vi "Disconnect.vi"(8 "error in (no error)":errorcluster, 10 "Disconnection list in":string, 11 "Consumer in":refnum<class "Consumer.lvclass">) -> (0 "error out":errorcluster, 3 "Consumer out":refnum<class "Consumer.lvclass">)   [LabVIEW 2020, in "%DEVICE% Messaging.lvlib" / "Consumer.lvclass"]
uses:
  Consumer.lvclass
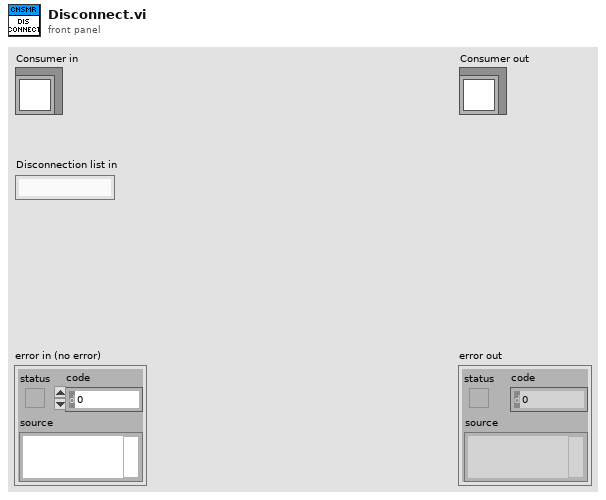
[diagram p1: front panel]
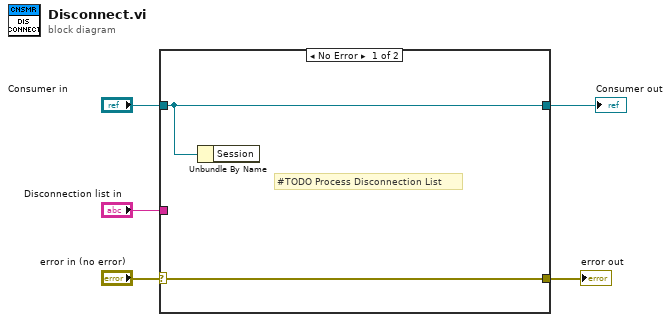
[diagram p0: block diagram]
diagram:
  n1 = case shown="No Error" "error in (no error)" {
    selector: "error in (no error)" -> [w6 w9]
    tunnel: [w6 w9] -> w3
    tunnel: [w7 w8] -> w2
    tunnel: "Consumer in" -> [w7 w8]
    tunnel: "Disconnection list in" -> [_ _]
    frame No Error {
      # "#TODO Process Disconnection List"
      n2 = Unbundle By Name(w7) -> ()  [unwired: 1 out]
    }
    frame Error {
    }
  }
  "error out" <- w3
  "Consumer out" <- w2
